vi "Utility - Set Project Tree & List Icons.vi"(8 "error in":errorcluster, 10 "MCListbox Refnum":refnum<vi>, 11 "Project Tree":T1) -> (0 "error out (Tree)":errorcluster, 2 "error out (MCList)":errorcluster)   [LabVIEW 2014]
doc: "::: VI Helpeks :::\nCopyright (c) 2000-2026 Konstantin Shifershteyn. All rights reserved."
uses:
  Project/VI Helpeks/_VIH Project Manager.llb/VIH Project Tree Typedef - Tree Item Type.ctl
  Project/VI Helpeks/_VIH Project Manager.llb/VIH Project Tree Typedef - Tree Refnum.ctl
panel:
  in  "ItemType":T2
  # "VI Helpeks\nCopyright (c) 2012-2026 Konstantin Shifershteyn"
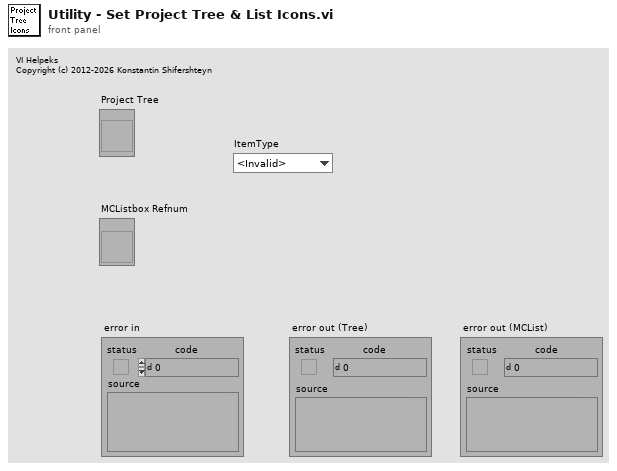
[diagram p1: front panel]
types:
  T1 = typedef "VIH Project Tree Typedef - Tree Refnum.ctl" = refnum<vi>
  T2 = typedef "VIH Project Tree Typedef - Tree Item Type.ctl" = enum32{"<Invalid>", "Project", "Proj Files", "Proj Rules", "File Group", "Rule Group", "Any File", "LV Func", ".mnu", ".mnu (dyn)", ".vi", ".vi (dyn)", ".vit", ".vit (dyn)", ".ctl", ".ctl (dyn)", ".ctt", ".ctt (dyn)", "polyVI", "polyVI (dyn)", "expVI", "expVI (dyn)", "HTML", "PolyVI Inst"}
  T3 = typedef "imagedata.ctl" = cluster{"image type":i32, "image depth":i32, "image":u8[], "mask":u8[], "colors":u32[], "Rectangle":cluster{"left":i16, "top":i16, "right":i16, "bottom":i16}}
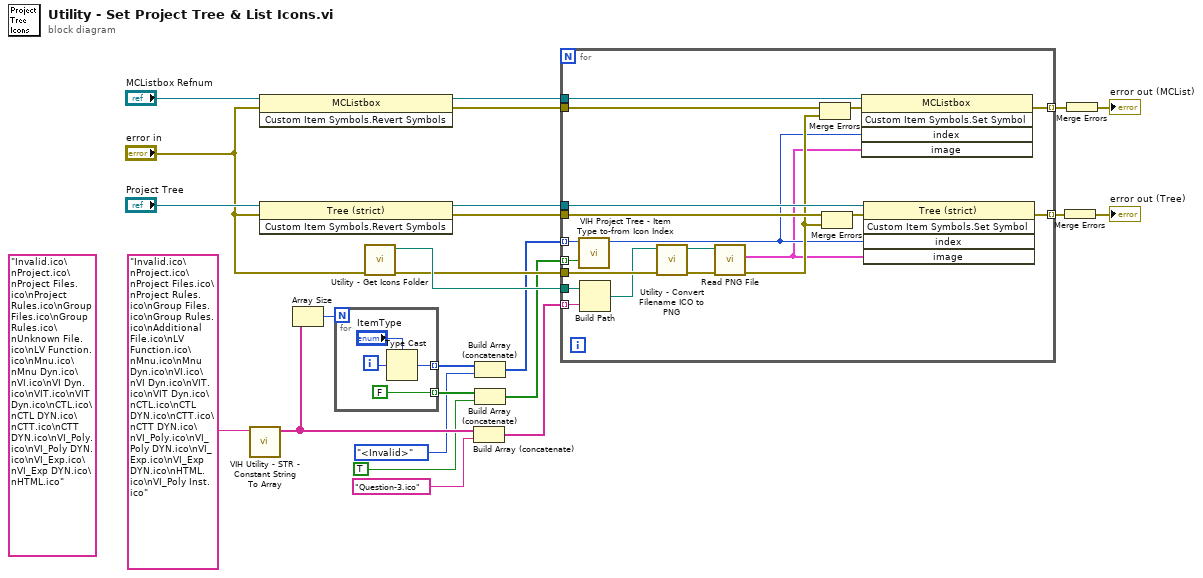
[diagram p0: block diagram]
diagram:
  (unwired) "Invalid.ico\nProject.ico\nProject Files.ico\nProject Rules.ico\nGroup Files.ico\nGroup Rules.ico\nUnknown File.ico\nLV Function.ico\nMnu.ico\nMnu Dyn.ico\nVI.ico\nVI Dyn.ico\nVIT.ico\nVIT Dyn.ico\nCTL.ico\nCTL DYN.ico\nCTT.ico\nCTT DYN.ico\nVI_Poly.ico\nVI_Poly DYN.ico\nVI_Exp.ico\nVI_Exp DYN.ico\nHTML.ico"
  n1 = call "VIH Utility - STR - Constant String To Array.vi"("String in"="Invalid.ico\nProject.ico\nProject Files.ico\nProject Rules.ico\nGroup Files.ico\nGroup Rules.ico\nAdditional File.ico\nLV Function.ico\nMnu.ico\nMnu Dyn.ico\nVI.ico\nVI Dyn.ico\nVIT.ico\nVIT Dyn.ico\nCTL.ico\nCTL DYN.ico\nCTT.ico\nCTT DYN.ico\nVI_Poly.ico\nVI_Poly DYN.ico\nVI_Exp.ico\nVI_Exp DYN.ico\nHTML.ico\nVI_Poly Inst.ico") -> ("Array out"=w18:string[])  [unwired: 10 in]
  n2 = invoke class="MCListbox" method="Custom Item Symbols.Revert Symbols"(reference="MCListbox Refnum", error in="error in") -> (reference out=w15:refnum<vi>, error out=w13:errorcluster)  [unwired: 1 in, 1 out]
  n3 = invoke class="Tree (strict)" method="Custom Item Symbols.Revert Symbols"(reference="Project Tree", error in="error in") -> (reference out=w23:T1, error out=w14:errorcluster)  [unwired: 1 in, 1 out]
  n4 = Array Size(array=w18) -> (size(s)=w20:i32)
  n5 = for {
    N: w20 -> [_]
    tunnel: [w27] -> w22 mode=indexing
    tunnel: [FALSE] -> w4 mode=indexing
    i -> [w28]
    n6 = Type Cast(type="ItemType", x=w28) -> (*(type *) &x=w27:T2)
  }
  n7 = call "Utility - Get Icons Folder.vi"("error in"="error in") -> ("error out"=w9:errorcluster, "Icons Folder"=w10:path)  [unwired: 9 in]
  n8 = Build Array (concatenate)(w18, "Question-3.ico") -> (w6:string[])
  n9 = Build Array (concatenate)(w22, VIH_Project_Tree_Typedef_-_Tree_Item_Type."<Invalid>" ("ItemType")) -> (w7:T2[])
  n10 = Build Array (concatenate)(w4, TRUE) -> (w1:bool[])
  n11 = for {
    tunnel: w23 -> [w46]
    tunnel: w7 -> [w45] mode=indexing
    tunnel: w10 -> [w44]
    tunnel: w6 -> [w43] mode=indexing
    tunnel: w9 -> [w41]
    tunnel: [w42] -> w21 mode=indexing
    tunnel: w15 -> [w40]
    tunnel: w14 -> [w38]
    tunnel: w13 -> [w37]
    tunnel: [w32] -> w12 mode=indexing
    tunnel: w1 -> [w31] mode=indexing
    n12 = call "VIH Project Tree - Item Type to-from Icon Index.vi"("Not found"=w31, "Item Type"=w45) -> ("Icon Index out"=w34:i32)  [unwired: 9 in]
    n13 = Build Path(base path=w44, name or relative path=w43) -> (appended path=w30:path)
    n14 = call "Utility - Convert Filename ICO to PNG.vi"("Path"=w30) -> ("Path 2"=w29:path)  [unwired: 10 in]
    n15 = call <vilib>:"Read PNG File.vi"("error in (no error)"=w41, "path to PNG file"=w29) -> ("error out"=w36:errorcluster, "image data"=w33:T3)  [unwired: 7 in, 1 out]
    n16 = Merge Errors(w37, w36) -> (w35:errorcluster)
    n17 = Merge Errors(w38, w36) -> (w39:errorcluster)
    n18 = invoke class="MCListbox" method="Custom Item Symbols.Set Symbol"(reference=w40, error in=w35, "index"=w34, "image"=w33) -> (error out=w32:errorcluster)  [unwired: 1 in, 4 out]
    n19 = invoke class="Tree (strict)" method="Custom Item Symbols.Set Symbol"(reference=w46, error in=w39, "index"=w34, "image"=w33) -> (error out=w42:errorcluster)  [unwired: 1 in, 4 out]
  }
  n20 = Merge Errors(w21) -> (→"error out (Tree)":errorcluster)
  n21 = Merge Errors(w12) -> (→"error out (MCList)":errorcluster)
